vi "ZM-HW-close.vi"(8 "error in (no error)":errorcluster, 11 "ZM-HW-hardware in":refnum<class "ZM-HW-hardware.lvclass">) -> (0 "error out":errorcluster, 3 "ZM-HW-hardware out":refnum<class "ZM-HW-hardware.lvclass">)   [LabVIEW 2020, in "ZM-HW-hardware.lvlib" / "ZM-HW-hardware.lvclass"]
doc: "Closes the hardware object: sets initialized = FALSE. This is where real hardware is put into a safe state; a child with real hardware overrides it and calls the parent."
uses:
  ZM-HW-hardware.lvclass
  ZM-HW-hardware.lvclass/ZM-HW-hardware.ctl
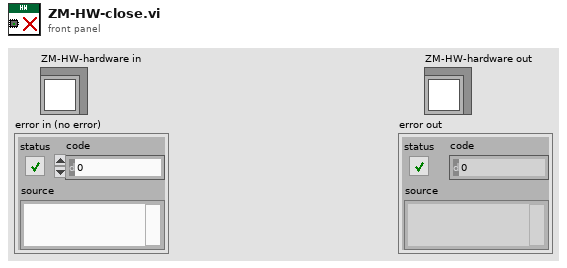
[diagram p1: front panel]
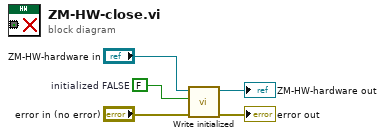
[diagram p0: block diagram]
diagram:
  w3 = FALSE  # initialized FALSE
  n1 = call "Write initialized.vi"("error in (no error)"="error in (no error)", "initialized"=w3, "ZM-HW-hardware in"="ZM-HW-hardware in") -> ("error out"=→"error out":errorcluster, "ZM-HW-hardware out"=→"ZM-HW-hardware out":refnum<class "ZM-HW-hardware.lvclass">)  [unwired: 7 in]
